vi "Rename lvlib.vi"(8 "error in":errorcluster, 9 "New Name":string, 10 "Library":string, 11 "IProject Manager in":refnum<class "Mock IProject Manager.lvclass">) -> (0 "error out":errorcluster, 3 "IProject Manager out":refnum<class "Mock IProject Manager.lvclass">)   [LabVIEW 2026, in "Mock IProject Manager.lvclass"]
doc: "Rename a library (.lvlib) to the provided new name. This VI renames both the project item and the file."
uses:
  Mock IProject Manager.lvclass
  C:/Program Files/National Instruments/LabVIEW 2026/vi.lib/Astemes/LMock/Mock.lvclass
  <vilib>/Astemes/LMock/Mock.lvclass
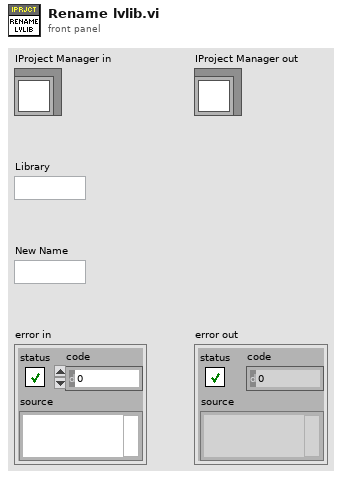
[diagram p1: front panel]
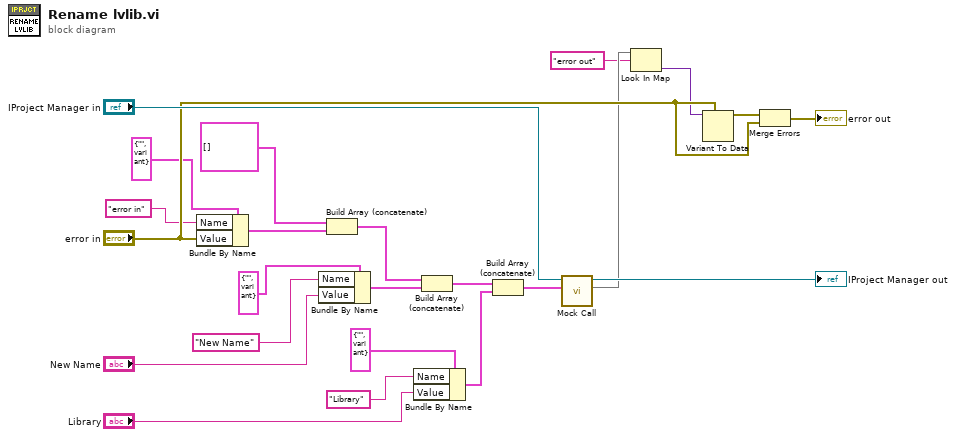
[diagram p0: block diagram]
diagram:
  n1 = Bundle By Name(cluster=cluster{"Name":string, "Value":variant} {"Name"="", "Value"=variant} ("element"), "Name"="error in", "Value"="error in") -> (w5:cluster{"Name":string, "Value":variant})
  n2 = Bundle By Name(cluster=cluster{"Name":string, "Value":variant} {"Name"="", "Value"=variant} ("element"), "Name"="New Name", "Value"="New Name") -> (w3:cluster{"Name":string, "Value":variant})
  n3 = Build Array (concatenate)(cluster{"Name":string, "Value":variant}[] [] ("Control Values"), w5) -> (w14:cluster{"Name":string, "Value":variant}[])
  n4 = Bundle By Name(cluster=cluster{"Name":string, "Value":variant} {"Name"="", "Value"=variant} ("element"), "Name"="Library", "Value"="Library") -> (w1:cluster{"Name":string, "Value":variant})
  n5 = Build Array (concatenate)(w14, w3) -> (w17:cluster{"Name":string, "Value":variant}[])
  n6 = Build Array (concatenate)(w17, w1) -> (w20:cluster{"Name":string, "Value":variant}[])
  n7 = call <vilib>:"Mock Call.vi"("Control Values"=w20, "Mock In"="IProject Manager in") -> ("Return Values"=w12:map{string, variant}, "Mock Out"=→"IProject Manager out":refnum<class "Mock IProject Manager.lvclass">)  [unwired: 8 in]
  n8 = Look In Map(map=w12, key="error out") -> (value=w10:variant)  [unwired: 1 in, 1 out]
  n9 = Variant To Data(type="error in", Variant=w10) -> (data=w9:errorcluster)  [unwired: 1 in, 1 out]
  n10 = Merge Errors(w9, "error in") -> (→"error out":errorcluster)
